vi "FuncVI-CPSpectrum.vi"(5 "InstanceRef":T2, 9 "arg list":T1[](array[typedef]) {"num" format="%.2f"}) -> (0 "error out":bool, 3 "result":T1 {"num" format="%.2f"})   [LabVIEW 2021]
doc: "::: CalcExpress Toolkit :::\nCopyright (c) 2000-2026 Konstantin Shifershteyn. All rights reserved."
uses:
  cetypes.llb/CalcExpress Function Argument Info.ctl
  cetypes.llb/CalcExpress Instance RefNum.ctl
  <vilib>/Analysis/NI_AALPro.lvlib
panel:
  in  "max arg num":i32=5
  in  "min arg num":i32=3
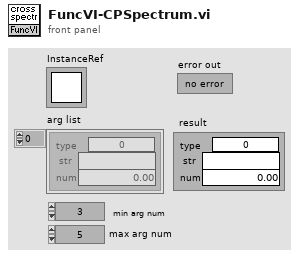
[diagram p1: front panel]
types:
  T1 = typedef "CalcExpress Function Argument Info.ctl" = cluster{"type":u32, "str":string, "num":dbl}
  T2 = typedef "CalcExpress Instance RefNum.ctl" = refnum<k1>
  T3 = enum8{"String", "DBL Number", "identifier", "1D Array of DBL", "2D Array of DBL", "CDB Number", "1D Array of CDB", "2D Array of CDB", "1D Array of String", "2D Array of String", "Unknown data type"}
  T4 = cluster{"index":i32, "type":enum8{"String", "DBL Number", "identifier", "1D Array of DBL", "2D Array of DBL", "CDB Number", "1D Array of CDB", "2D Array of CDB", "Unknown data type"}, "default num":dbl, "default str":string}[]
  T5 = typedef "VarMan Variable Context Handle.ctl" = i32
  T6 = cluster{"type":enum8{"String", "DBL Number", "identifier", "1D Array of DBL", "2D Array of DBL", "CDB Number", "1D Array of CDB", "2D Array of CDB", "1D Array of String", "2D Array of String", "Unknown data type"}, string, "df":dbl}
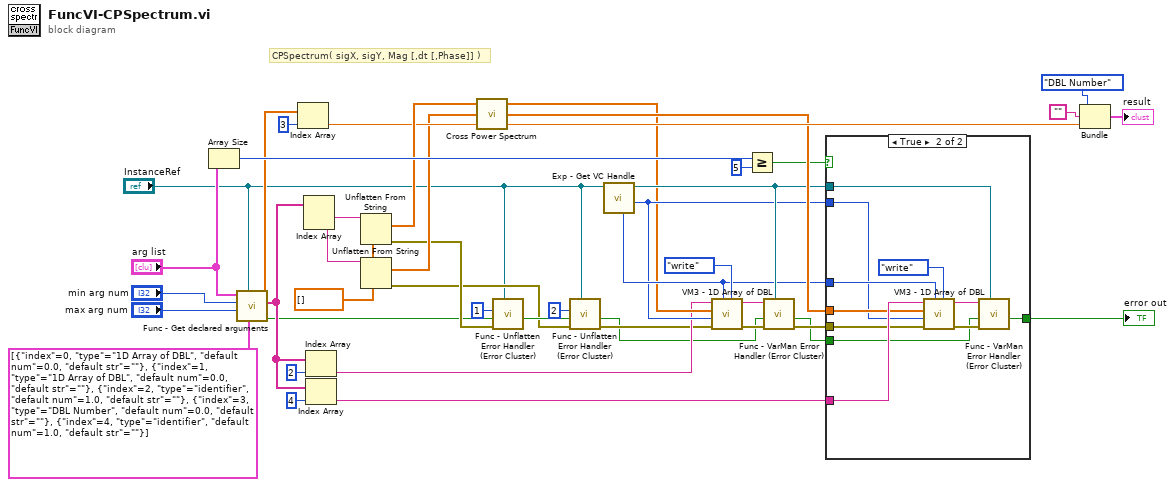
[diagram p0: block diagram]
diagram:
  w24 = dbl[] [] ("value out")
  # "CPSpectrum( sigX, sigY, Mag [,dt [,Phase]] )"
  n1 = Array Size(array="arg list") -> (size(s)=w37:i32)
  n2 = call "Func - Get declared arguments.vi"("arg descriptors"=T4 [{"index"=0, "type"=enum."1D Array of DBL", "default num"=0.0, "default str"=""}, {"index"=1, "type"=enum."1D Array of DBL", "default num"=0.0, "default str"=""}, {"index"=2, "type"=enum."identifier", "default num"=1.0, "default str"=""}, {"index"=3, "type"=enum."DBL Number", "default num"=0.0, "default str"=""}, {"index"=4, "type"=enum."identifier", "default num"=1.0, "default str"=""}] ("args descriptors"), "InstanceRef"="InstanceRef", "max arg num"="max arg num", "min arg num"="min arg num", "arg list"="arg list") -> ("error out"=w3:bool, "str list"=w25:string[], "num list"=w26:dbl[])  [unwired: 3 in, 1 out]
  n3 = Index Array(array=w26, index=3) -> (element=w27:dbl)
  n4 = Index Array(array=w25) -> (element #1=w30:string, element #2=w4:string)  [unwired: 2 in]
  n5 = Index Array(array=w25, index=2) -> (element=w9:string)
  n6 = Index Array(array=w25, index=4) -> (element=w32:string)
  n7 = Unflatten From String(type=w24, binary string=w30) -> (value=w29:dbl[], error out=w7:errorcluster)  [unwired: 3 in, 1 out]
  n8 = Unflatten From String(type=w24, binary string=w4) -> (value=w23:dbl[], error out=w6:errorcluster)  [unwired: 3 in, 1 out]
  n9 = call <vilib>:"Cross Power Spectrum.vi"("dt"=w27, "Signal Y (V)"=w23, "Signal X (V)"=w29) -> ("df"=w42:dbl, "Cross Power XY Spectrum Phase (radians)"=w41:dbl[], "Cross Power XY Spectrum Mag (V^2rms)"=w11:dbl[])
  n10 = call "Func - Unflatten Error Handler (Error Cluster).vi"("InstanceRef"="InstanceRef", "Unflatten Error Cluster"=w7, "error status before"=w3, "argument number"=1) -> ("error status out"=w18:bool)  [unwired: 5 in, 2 out]
  n11 = call "Func - Unflatten Error Handler (Error Cluster).vi"("InstanceRef"="InstanceRef", "Unflatten Error Cluster"=w6, "error status before"=w18, "argument number"=2) -> ("Error Cluster out"=w8:errorcluster, "error status out"=w1:bool)  [unwired: 5 in, 1 out]
  n12 = call "Exp - Get VC Handle.vi"("InstanceRef"="InstanceRef") -> ("writer ID"=w12:u32, "dup InstanceRef"=w14:T2, "VC Handle"=w13:T5)  [unwired: 5 in, 1 out]
  n13 = call "VM3 - 1D Array of DBL.vi"("cmd (read)"=enum16{"create", "destroy", "write", "read"}."write", "VC Handle"=w13, "error in"=w8, "writer ID"=w12, "value in"=w11, "name_spec"=w9) -> ("error out"=w10:errorcluster, "dup name_spec"=w16:string)  [unwired: 2 in, 2 out]
  n14 = Greater Or Equal?(x=w37, y=5) -> (x >= y?=w39:bool)
  n15 = call "Func - VarMan Error Handler (Error Cluster).vi"("InstanceRef"=w14, "VarMan VI error in"=w10, "error status before"=w1, "var name"=w16) -> ("error out"=w15:errorcluster, "FuncVI error out"=w5:bool)  [unwired: 5 in, 1 out]
  n16 = case shown="True" w39 {
    tunnel: w5 -> [w45 w46]
    tunnel: w41 -> [_ w49]
    tunnel: [w45 w53] -> w40
    tunnel: w32 -> [_ w50]
    tunnel: w14 -> [_ w52]
    tunnel: w13 -> [_ w51]
    tunnel: w12 -> [_ w48]
    tunnel: w15 -> [_ w47]
    frame False {
    }
    frame True {
      n17 = call "VM3 - 1D Array of DBL.vi"("cmd (read)"=enum16{"create", "destroy", "write", "read"}."write", "VC Handle"=w51, "error in"=w47, "writer ID"=w48, "value in"=w49, "name_spec"=w50) -> ("error out"=w56:errorcluster, "dup name_spec"=w55:string)  [unwired: 2 in, 2 out]
      n18 = call "Func - VarMan Error Handler (Error Cluster).vi"("InstanceRef"=w52, "VarMan VI error in"=w56, "error status before"=w46, "var name"=w55) -> ("FuncVI error out"=w53:bool)  [unwired: 5 in, 2 out]
    }
  }
  "error out" <- w40
  n19 = Bundle("type"=T3."DBL Number", "", "df"=w42) -> (→"result":T6)  [unwired: 1 in]
